vi "Stop Motor.vi"(8 "error in (no error)":errorcluster, 10 "Target":enum16{"Mast", "Turn Table"}(ring), 11 "CO3000 in":refnum<class "CO3000.lvclass">) -> (0 "error out":errorcluster, 3 "CO3000 out":refnum<class "CO3000.lvclass">)   [LabVIEW 2023, in "Turn Table and Mast.lvlib" / "CO3000.lvclass"]
uses:
  CO3000.lvclass
  CO3000.lvclass/CO3000.ctl
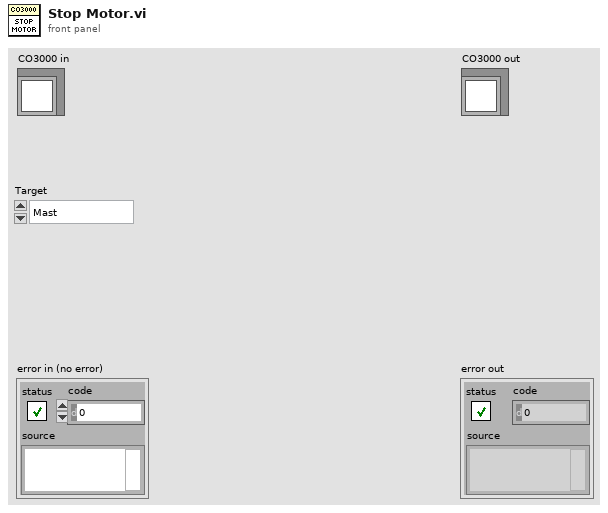
[diagram p1: front panel]
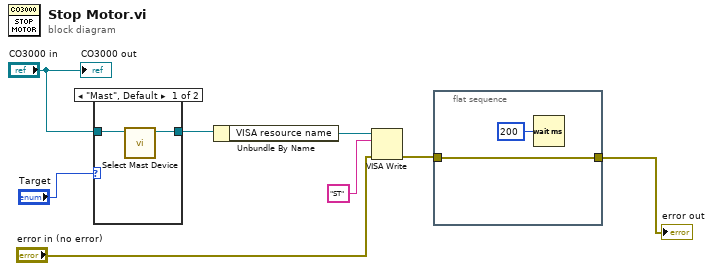
[diagram p0: block diagram]
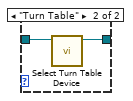
[diagram p2: hidden frame]
diagram:
  n1 = case shown="\"Mast\", Default" "Target" {
    tunnel: "CO3000 in" -> [w10 w12]
    tunnel: [w9 w11] -> w2
    frame "Mast", Default {
      n2 = call "Select Mast Device.vi"("CO3000 in"=w10) -> ("CO3000 out"=w9:refnum<class "CO3000.lvclass">)  [unwired: 9 in, 1 out]
    }
    frame "Turn Table" {
      n3 = call "Select Turn Table Device.vi"("CO3000 in"=w12) -> ("CO3000 out"=w11:refnum<class "CO3000.lvclass">)  [unwired: 9 in, 1 out]
    }
  }
  n4 = Unbundle By Name(w2) -> ("VISA resource name"=w8:refnum<visa-resource-name>)
  n5 = VISA Write(VISA resource name=w8, write buffer="ST", error in (no error)="error in (no error)") -> (error out=w6:errorcluster)  [unwired: 2 out]
  n6 = flat-sequence {
    tunnel: w6 -> [w13]
    tunnel: [w13] -> w5
    frame #0 {
      n7 = Wait (ms)(milliseconds to wait=u32 200) -> ()  [unwired: 1 out]
    }
  }
  "error out" <- w5
  "CO3000 out" <- "CO3000 in"
